vi "Temperature Monitor.vi"() -> ()   [LabVIEW 2026]
doc: "Reads a temperature, compares it against an alarm threshold and reports a status string plus a boolean alarm flag. Self-contained: primitives only, no subVI calls, so it passes the generator's self-containment rule."
panel:
  out "Alarm":bool
  out "Status":string="Normal"
  in  "Alarm Threshold":dbl=80.0
  in  "Temperature":dbl=25.0
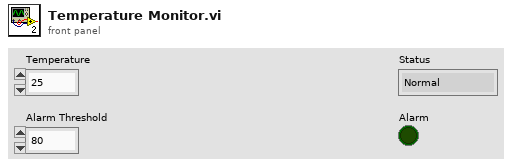
[diagram p1: front panel]
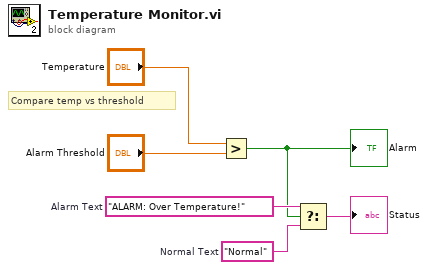
[diagram p0: block diagram]
diagram:
  w3 = "Normal"  # Normal Text
  w4 = "ALARM: Over Temperature!"  # Alarm Text
  # "Compare temp vs threshold"
  n1 = Greater?(x="Temperature", y="Alarm Threshold") -> (0:w1:bool)
  "Alarm" <- w1
  n2 = Select(t=w4, s=w1, f=w3) -> (s? t:f=→"Status":string)
